vi "VIH HelpGen - Build CHM File.vi"(8 "error in":errorcluster, 9 "Compile CHM file":bool, 10 "Create HHP file":bool, 11 "Project Tree":T1) -> (0 "error out":errorcluster, 1 "CHM File path":path, 2 "HHP File path":path, 3 "dup Project Tree":T1)   [LabVIEW 2014]
doc: "::: VI Helpeks :::\nCopyright (c) 2000-2026 Konstantin Shifershteyn. All rights reserved."
uses:
  _VIH Project Manager.llb/VIH Project Tree Typedef - Tree Refnum.ctl
panel:
  # "VI Helpeks\nCopyright (c) 2012-2026 Konstantin Shifershteyn"
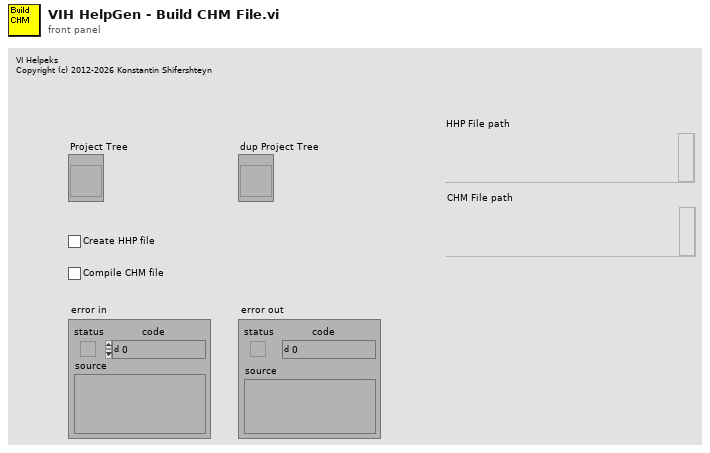
[diagram p1: front panel]
types:
  T1 = typedef "VIH Project Tree Typedef - Tree Refnum.ctl" = refnum<vi>
  T2 = enum16{"nop", "Init", "Run-HHP", "Run-CHM", "Run-INFO"}
  T3 = typedef "VIH - CHM Project - HHP Generation Params Cluster.ctl" = cluster{"HHP_Template":enum16{"default", "custom"}, "HHP_Template_CustomPath":path, "HHP_Target":enum16{"default", "custom"}, "HHP_Target_CustomPath":path, "HHP_CreateTOC":bool, "HHP_CreateIDX":bool, "HHP_DefaultTopic":enum16{"auto", "custom"}, "HHP_DefaultTopic_CustomPath":path, "CHM_Filename":path, "HHP_AutoBuild":bool, "CHM_AutoBuild":bool}
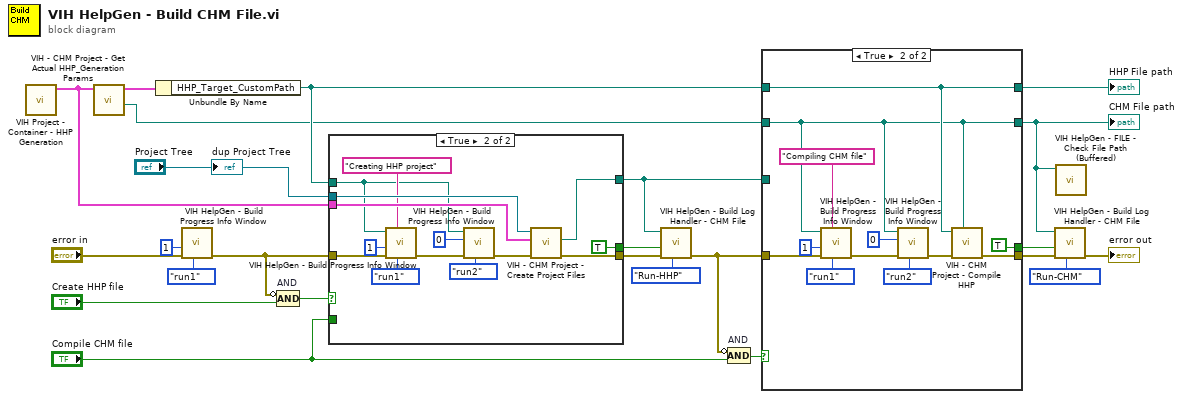
[diagram p0: block diagram]
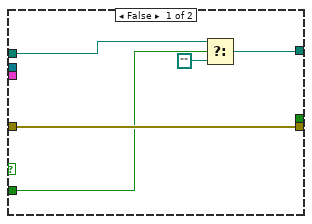
[diagram p3: hidden frame]
diagram:
  n1 = call "VIH Project - Container - HHP Generation.vi"() -> ("HHP_Generation out"=w23:T3)  [unwired: 11 in]
  n2 = call "VIH - CHM Project - Get Actual HHP_Generation Params.vi"("HHP_Generation"=w23) -> ("CHM File Absolute Path"=w16:path, "HHP_Generation out"=w24:T3)  [unwired: 8 in, 1 out]
  n3 = Unbundle By Name(w24) -> ("HHP_Target_CustomPath"=w22:path)
  n4 = call "VIH HelpGen - Build Progress Info Window.vi"("Mode (run1)"=enum16{"start", "stop", "run1", "run2"}."run1", "error in"="error in", "# steps"=1) -> ("error out"=w7:errorcluster)  [unwired: 8 in]
  n5 = Compound Arithmetic op=AND "AND"(invert w7, "Create HHP file") -> (w5:bool)
  n6 = case shown="True" w5 {
    tunnel: "Project Tree" -> [_ w43]
    tunnel: w23 -> [_ w42]
    tunnel: w7 -> [w29 w40]
    tunnel: [w29 w32] -> w11
    tunnel: w22 -> [w28 w36]
    tunnel: [w27 w31] -> w8
    tunnel: [_ TRUE] -> w9
    tunnel: "Compile CHM file" -> [w25 _]
    frame False {
      n7 = Select(t=w28, s=w25, f=path "") -> (s? t:f=w27:path)
    }
    frame True {
      n8 = call "VIH HelpGen - Build Progress Info Window.vi"("Mode (run1)"=enum16{"start", "stop", "run1", "run2"}."run1", "Message"="Creating HHP project", "error in"=w40, "# steps"=1, "Cur path"=w36) -> ("error out"=w34:errorcluster)  [unwired: 6 in]
      n9 = call "VIH HelpGen - Build Progress Info Window.vi"("Mode (run1)"=enum16{"start", "stop", "run1", "run2"}."run2", "error in"=w34, "step idx"=0, "Cur path"=w36) -> ("error out"=w33:errorcluster)  [unwired: 7 in]
      n10 = call "VIH - CHM Project - Create Project Files.vi"("error in"=w33, "HHP_Generation"=w42, "Project Tree"=w43) -> ("error out"=w32:errorcluster, "Target HHP File"=w31:path)  [unwired: 6 in, 1 out]
    }
  }
  n11 = call "VIH HelpGen - Build Log Handler - CHM File.vi"("cmd (nop)"=T2."Run-HHP", "error in"=w11, "File Built"=w9, "File Path 1"=w8) -> ("error out"=w10:errorcluster)  [unwired: 5 in, 2 out]
  n12 = Compound Arithmetic op=AND "AND"(invert w10, "Compile CHM file") -> (w13:bool)
  n13 = case shown="True" w13 {
    tunnel: w10 -> [w45 w47]
    tunnel: w16 -> [_ w48]
    tunnel: [w45 w50] -> w15
    tunnel: w22 -> [_ w49]
    tunnel: [_ w48] -> w4
    tunnel: [w44 w49] -> w17
    tunnel: w8 -> [w44 _]
    tunnel: [_ TRUE] -> w12
    frame False {
    }
    frame True {
      n14 = call "VIH HelpGen - Build Progress Info Window.vi"("Mode (run1)"=enum16{"start", "stop", "run1", "run2"}."run1", "Message"="Compiling CHM file", "error in"=w47, "# steps"=1, "Cur path"=w48) -> ("error out"=w52:errorcluster)  [unwired: 6 in]
      n15 = call "VIH HelpGen - Build Progress Info Window.vi"("Mode (run1)"=enum16{"start", "stop", "run1", "run2"}."run2", "error in"=w52, "step idx"=0, "Cur path"=w48) -> ("error out"=w51:errorcluster)  [unwired: 7 in]
      n16 = call "VIH - CHM Project - Compile HHP.vi"("CHM File Path"=w48, "error in"=w51, "HHP File Path"=w49) -> ("error out"=w50:errorcluster)  [unwired: 6 in, 2 out]
    }
  }
  "HHP File path" <- w17
  "CHM File path" <- w4
  n17 = call "VIH HelpGen - Build Log Handler - CHM File.vi"("cmd (nop)"=T2."Run-CHM", "error in"=w15, "File Built"=w12, "File Path 1"=w4) -> ("error out"=→"error out":errorcluster)  [unwired: 5 in, 2 out]
  n18 = call "VIH HelpGen - FILE - Check File Path (Buffered).vi"("File Path"=w4) -> ()  [unwired: 9 in, 2 out]
  "dup Project Tree" <- "Project Tree"
